vi "CreatCursor (SubVI).vi"(8 "error in (no error)":errorcluster, 10 "Array in":dbl[][](array[numeric]), 11 "XYGraph in":refnum<vi>) -> (2 "Array out":cluster{"X":dbl[], "Y":dbl[]}[](array[cluster]))   [LabVIEW 2017]
uses:
  <vilib>/Utility/miscctls.llb/LVCursorListTypeDef.ctl
panel:
  out "error out":errorcluster
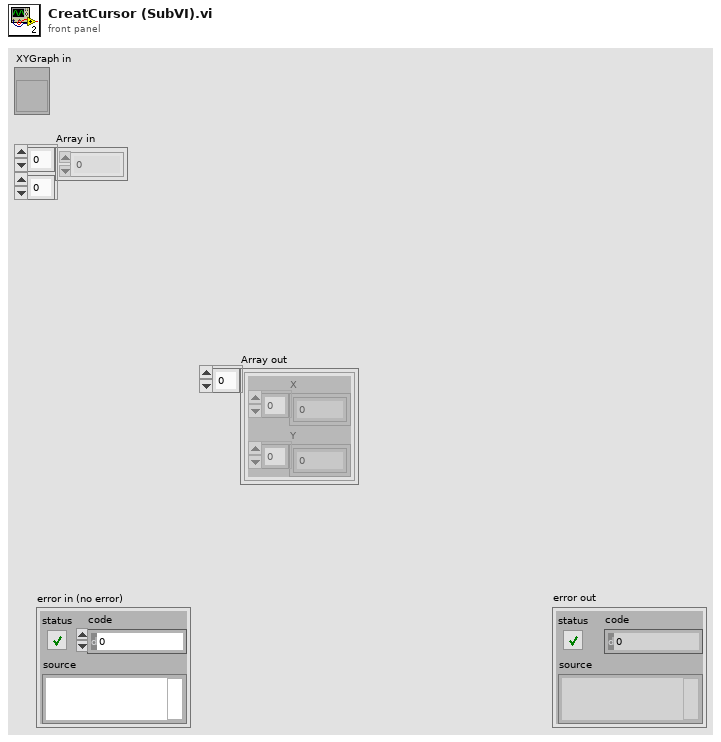
[diagram p1: front panel]
types:
  T1 = typedef "LVCursorListTypeDef.ctl" = cluster{"Name":string, "Color":u32, "Style":u8, "Point Style":u8, "Name Visible":bool, "Allow Drag":bool, "Cursor Mode":u32, "Plot":i32, "Index":i32, "Position":cluster{"X":dbl, "Y":dbl}, "X Scale":u32, "Y Scale":u32, "Watch Plots":i32[], "Watch All Plots":bool, "Plot Area":i32, "Label Offset":cluster{"X":dbl, "Y":dbl}}[]
  T2 = cluster{"Name":string, "Color":u32, "Style":u8, "Point Style":u8, "Name Visible":bool, "Allow Drag":bool, "Cursor Mode":u32, "Plot":i32, "Index":i32, "Position":cluster{"X":dbl, "Y":dbl}, "X Scale":u32, "Y Scale":u32, "Watch Plots":i32[], "Watch All Plots":bool, "Plot Area":i32, "Label Offset":cluster{"X":dbl, "Y":dbl}}
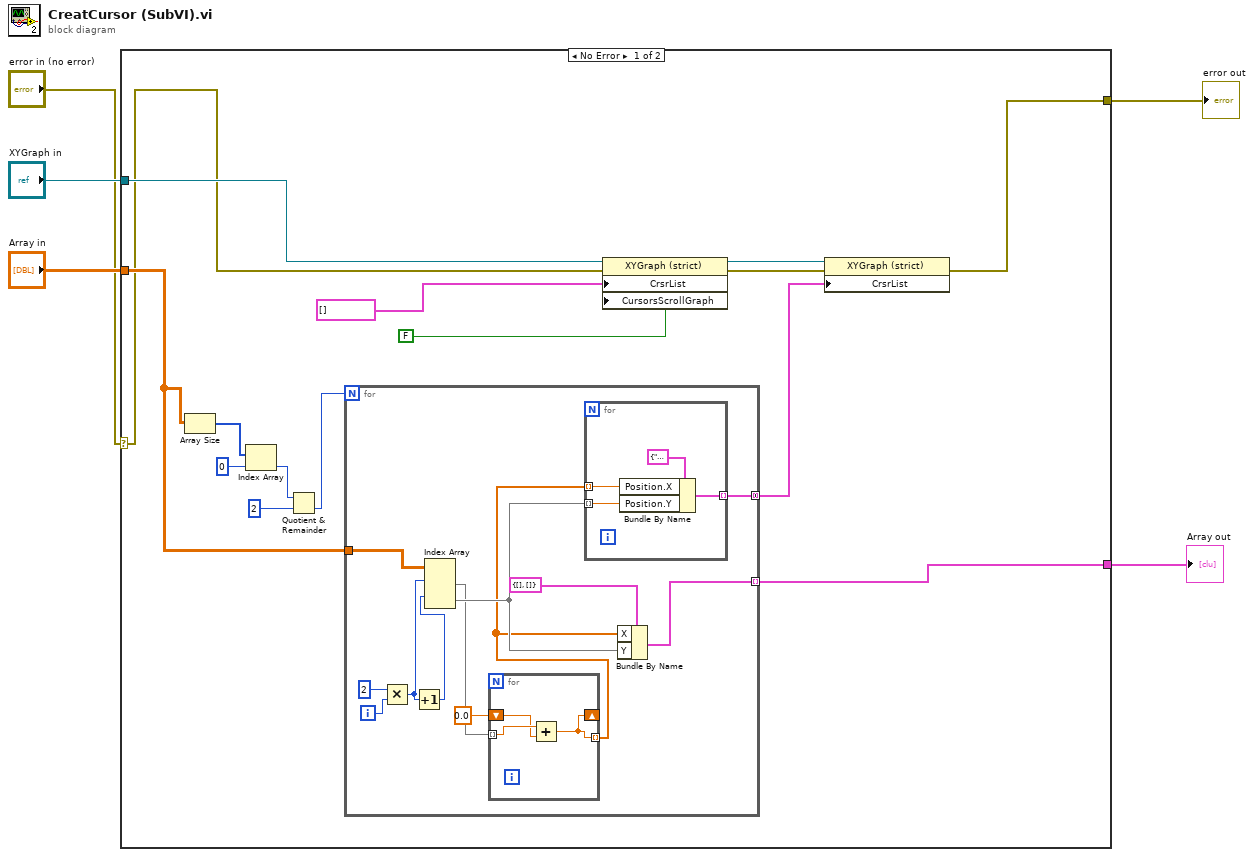
[diagram p0: block diagram]
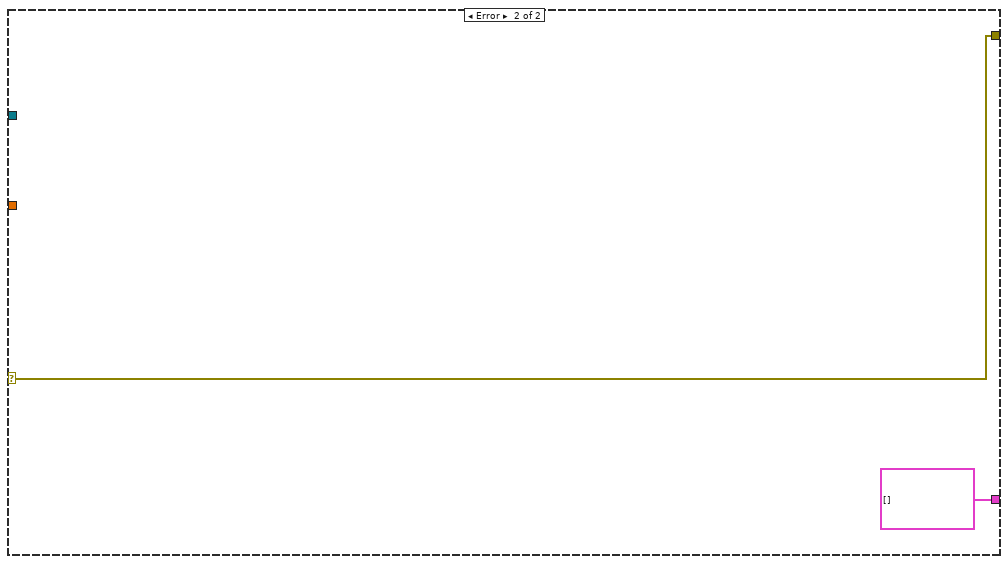
[diagram p2: hidden frame]
diagram:
  n1 = case shown="No Error" "error in (no error)" {
    selector: "error in (no error)" -> [w7 w41]
    tunnel: "Array in" -> [w20 _]
    tunnel: [w18 cluster{"X":dbl[], "Y":dbl[]}[] []] -> w4
    tunnel: "XYGraph in" -> [w9 _]
    tunnel: [w12 w41] -> w2
    frame No Error {
      n2 = Array Size(array=w20) -> (size(s)=w13:i32[])
      n3 = Index Array(array=w13, index=0) -> (element=w15:i32)
      n4 = Quotient & Remainder(x=w15, y=2) -> (floor(x/y)=w19:i32)  [unwired: 1 out]
      n5 = for {
        N: w19 -> [_]
        tunnel: w20 -> [w32]
        tunnel: [w27] -> w18 mode=indexing
        tunnel: [w26] -> w17 mode=concatenating
        i -> [w31]
        n6 = Multiply(x=2, y=w31) -> (x*y=w29:i32)
        n7 = Increment(x=w29) -> (x+1=w28:i32)
        n8 = Index Array(array=w32, index (row) #1=w29, index (row) #2=w28) -> (element #1=w23:dbl[], element #2=w24:dbl[])  [unwired: 2 in]
        n9 = for {
          shift-right: [w33] -> _
          shift-left: 0.0 -> [w34]
          tunnel: w23 -> [w35] mode=indexing
          tunnel: [w33] -> w21 mode=indexing
          n10 = Add(x=w35, y=w34) -> (x+y=w33:dbl)
        }
        n11 = for {
          tunnel: w21 -> [w38] mode=indexing
          tunnel: w24 -> [w37] mode=indexing
          tunnel: [w36] -> w26 mode=indexing
          n12 = Bundle By Name(cluster=T2 {"Name"="upper limit 0", "Color"=16777216, "Style"=0, "Point Style"=13, "Name Visible"=FALSE, "Allow Drag"=TRUE, "Cursor Mode"=0, "Plot"=0, "Index"=4, "Position"={"X"=0.0, "Y"=10.0}, "X Scale"=0, "Y Scale"=0, "Watch Plots"=[], "Watch All Plots"=FALSE, "Plot Area"=0, "Label Offset"={"X"=1.8341968911917097, "Y"=18.604651162790695}}, "Position.X"=w38, "Position.Y"=w37) -> (w36:T2)
        }
        n13 = Bundle By Name(cluster=cluster{"X":dbl[], "Y":dbl[]} {"X"=[], "Y"=[]}, "X"=w21, "Y"=w24) -> (w27:cluster{"X":dbl[], "Y":dbl[]})
      }
      n14 = property on="Property Node" class="XYGraph (strict)"(reference=w9, error in=w7, "CrsrList"=T1 [] ("Cursor List"), "CursorsScrollGraph"=FALSE ("Cursors Scroll Graph")) -> (reference out=w8:refnum<vi>, error out=w6:errorcluster)
      n15 = property on="Property Node" class="XYGraph (strict)"(reference=w8, error in=w6, "CrsrList"=w17) -> (error out=w12:errorcluster)  [unwired: 1 out]
    }
    frame Error {
    }
  }
  "Array out" <- w4
  "error out" <- w2
